vi "ingest.trigger_file_ingest-new_dataset.vi"(5 "prefixTreeDelimiter":string, 6 "Properties and Labels":T1, 7 "Timestamp Metadata":refnum<class "timestampMetadata.lvclass">, 8 "error in":errorcluster, 9 "Title and Description":cluster{"Title":string, "Description":string}, 10 "S3 Path to File":string, 11 "Nominal Client in":refnum<class "Nominal Client.lvclass">) -> (0 "error out":errorcluster, 2 "Information":T2, 3 "Nominal Client out":refnum<class "Nominal Client.lvclass">, 4 "Response":string)   [LabVIEW 2020, in "Nominal Client.lvclass"]
doc: "<b> DEPRECIATED METHOD: Use Ingest All.vi for new projects </b>\n\nTriggers an ingest job of a new file, allowing either creating a new dataset or uploading to an existing one."
uses:
  Nominal Client.lvclass
  timestampMetadata/timestampMetadata.lvclass
  Nominal Client.lvclass/Nominal Client.ctl
  4b965f09-dc68-4d5e-a5c1-32d476accfd4.vi
  ae647589-d40a-40ab-8bd3-12ed03615a29.vi
  49ecdc87-d06e-40b5-807d-cfeea5b09dd4.vi
  trace.payload_received.vi
  error.vi
  trace.payload_sent.vi
  create.authorization_header.vi
  trace.calling_method.vi
  error.vi/859f8e04-e495-489b-b5b4-7ac163f56130.vi
  <vilib>/JDP Science/JDP Science Common Utilities/Trim Whitespace__JDP.vi
  <vilib>/AdvancedString/1D String Array to Delimited String.vi
  api_token.get.vi
  <vilib>/JDP Science/JSONtext/Variant to JSON Text.vi
  <vilib>/JDP Science/JSONtext/Array of Variants to JSON Object.vi
  <vilib>/JDP Science/JSONtext/Set Item.vi
  <vilib>/Utility/libraryn.llb/Get File Extension.vi
  log_file.write.vi
  <vilib>/JDP Science/JSONtext/Get all Object Items.vi
  <vilib>/Utility/error.llb/Error Cluster From Error Code.vi
  <vilib>/JDP Science/JSONtext/JSON text to Variant.vi
  <vilib>/JDP Science/JSONtext/LVClass Serializer/JSONtext LVClass Serializer.lvclass
  <vilib>/addons/_JKI.lib/REST Client/classes/Response Headers/Response Headers.lvclass
  <vilib>/addons/_JKI.lib/REST Client/classes/REST Client/REST Client.lvclass
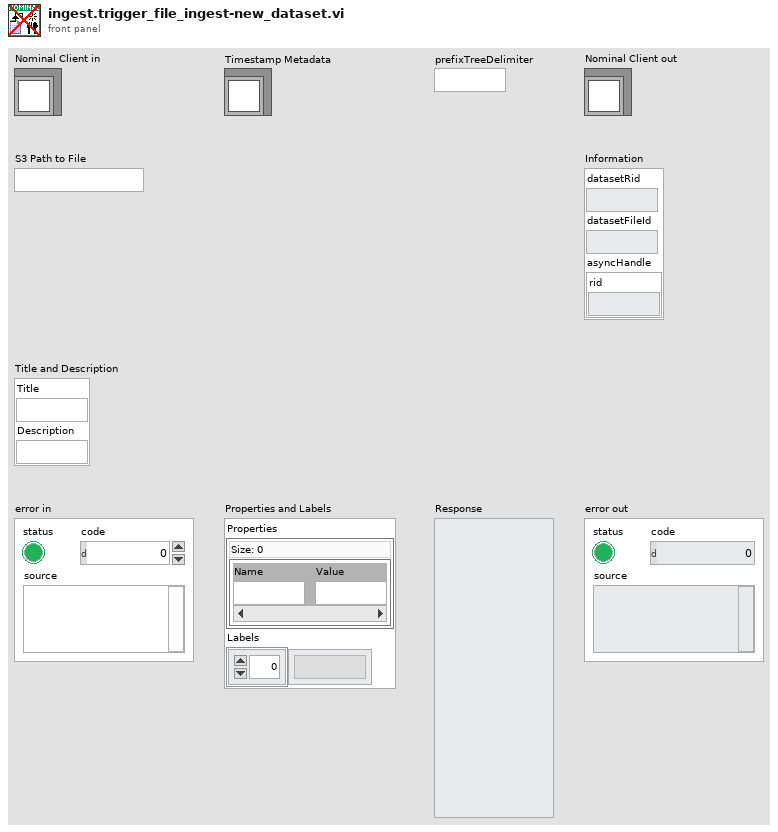
[diagram p1: front panel]
types:
  T1 = cluster{"Properties":map{string, string}, "Labels":string[]}
  T2 = cluster{"datasetRid":string, "datasetFileId":string, "asyncHandle":cluster{"rid":string}}
  T3 = cluster{"type":string, "s3":cluster{"path":string}}
  T4 = cluster{"type":string, "newDataset":cluster{"properties":string, "labels":string[], "datasetName":string, "datasetDescription":string, "channelConfig":cluster{"prefixTreeDelimiter":string}}}
  T5 = cluster{"source":cluster{"type":string, "s3":cluster{"path":string}}, "destination":cluster{"type":string, "newDataset":cluster{"properties":string, "labels":string[], "datasetName":string, "datasetDescription":string, "channelConfig":cluster{"prefixTreeDelimiter":string}}}, "sourceMetadata":cluster{"timestampMetadata":string}}
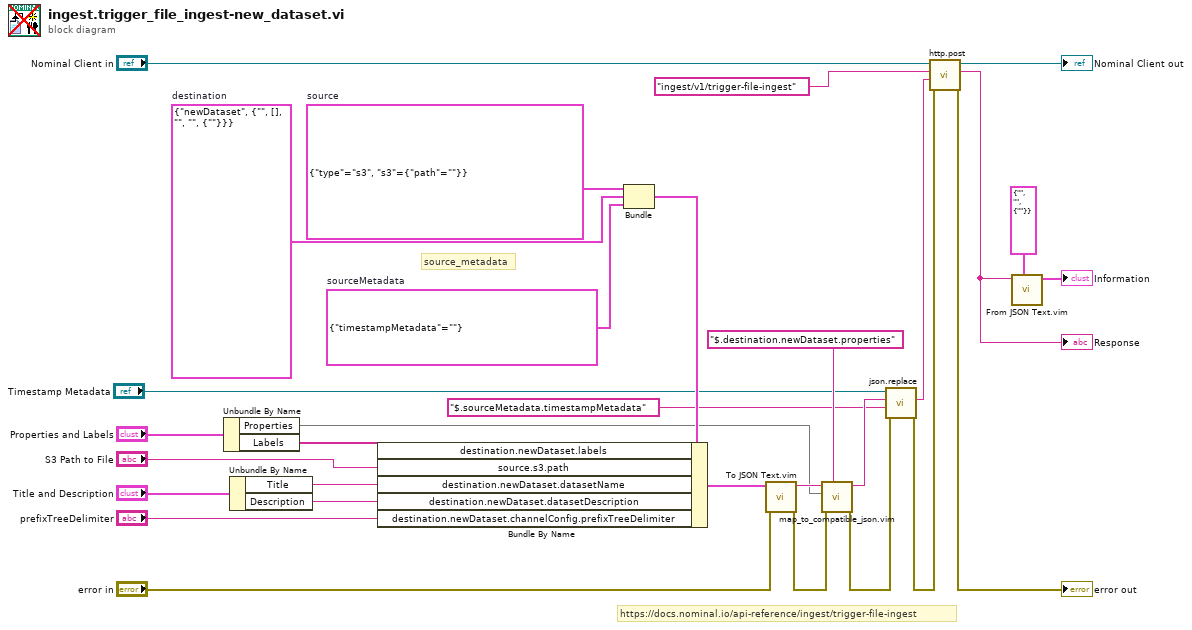
[diagram p0: block diagram]
diagram:
  w3 = cluster{"timestampMetadata":string} {"timestampMetadata"=""}  # sourceMetadata
  w26 = T3 {"type"="s3", "s3"={"path"=""}}  # source
  w27 = T4 {"type"="newDataset", "newDataset"={"properties"="", "labels"=[], "datasetName"="", "datasetDescription"="", "channelConfig"={"prefixTreeDelimiter"=""}}}  # destination
  # "source_metadata"
  # "https://docs.nominal.io/api-reference/ingest/trigger-file-ingest"
  n1 = Unbundle By Name("Properties and Labels") -> ("Properties"=w14:map{string, string}, "Labels"=w15:string[])
  n2 = Unbundle By Name("Title and Description") -> ("Title"=w11:string, "Description"=w12:string)
  n3 = Bundle("source"=w26, "destination"=w27, "sourceMetadata"=w3) -> (w25:T5)  [unwired: 1 in]
  n4 = Bundle By Name(cluster=w25, "destination.newDataset.labels"=w15, "source.s3.path"="S3 Path to File", "destination.newDataset.datasetName"=w11, "destination.newDataset.datasetDescription"=w12, "destination.newDataset.channelConfig.prefixTreeDelimiter"="prefixTreeDelimiter") -> (w24:T5)
  n5 = call "To JSON Text.vim"("error in (no error)"="error in", "Anything"=w24) -> ("error out"=w17:errorcluster, "<JSON>"=w18:string)  [unwired: 8 in]
  n6 = call "map_to_compatible_json.vim"("JSON Path"="$.destination.newDataset.properties" ("Data Name"), "error in"=w17, "Map"=w14, "JSON in"=w18) -> ("error out"=w5:errorcluster, "JSON out"=w7:string)  [unwired: 6 in]
  n7 = call "json.replace.vi"("error in"=w5, "Object To Update"="$.sourceMetadata.timestampMetadata" ("Object Name"), "JSON in"=w7, "timestampMetadata in"="Timestamp Metadata") -> ("error out"=w4:errorcluster, "JSON out"=w6:string)  [unwired: 5 in, 1 out]
  n8 = call "http.post.vi"("error in"=w4, "Request body"=w6, "Path"="ingest/v1/trigger-file-ingest", "Nominal Client in"="Nominal Client in") -> ("error out"=→"error out":errorcluster, "Response"=w1:string, "Nominal Client out"=→"Nominal Client out":refnum<class "Nominal Client.lvclass">)  [unwired: 4 in, 1 out]
  "Response" <- w1
  n9 = call "From JSON Text.vim"("Data Type and Default Value"=T2 {"datasetRid"="", "datasetFileId"="", "asyncHandle"={"rid"=""}} ("Information"), "JSON"=w1) -> ("Data out"=→"Information":T2)  [unwired: 8 in, 1 out]
